vi "snapPoint.vi"(0 "reference":refnum<class "Grid.lvclass">, 1 "point2D":T1 {"y" format="%.2f"; "x" format="%.2f"}, 5 "error in (no error)":errorcluster) -> (14 "reference out":refnum<class "Grid.lvclass">, 15 "point2D 2":T1 {"y" format="%.2f"; "x" format="%.2f"}, 19 "error out":errorcluster)   [LabVIEW 2020, in "Grid.lvclass"]
doc: "public void snap(Point2D p)"
uses:
  <resource>/Framework/Providers/Open_GDS/UML/Grid_class/Grid.lvclass
  <resource>/Framework/Providers/Open_GDS/UML/General/Point/Point Point2D.ctl
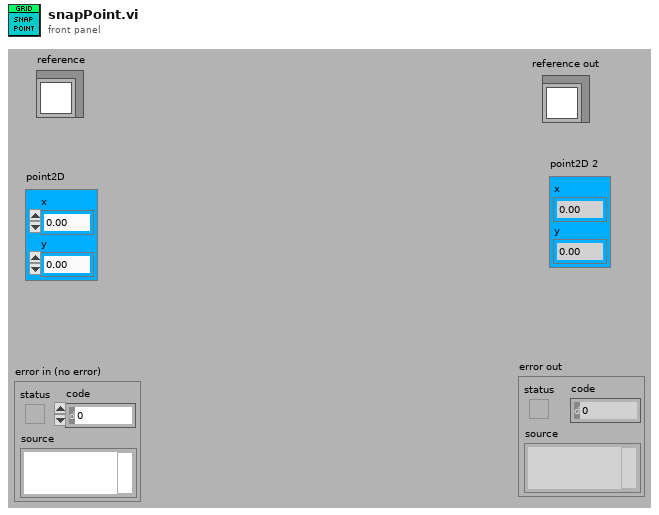
[diagram p1: front panel]
types:
  T1 = typedef "Point Point2D.ctl" = cluster{"x":dbl, "y":dbl}
  T2 = typedef "Grid.lvclass/ObjectAttributes.ctl" = cluster{"gridX":dbl, "gridY":dbl, "gridColor":u32}
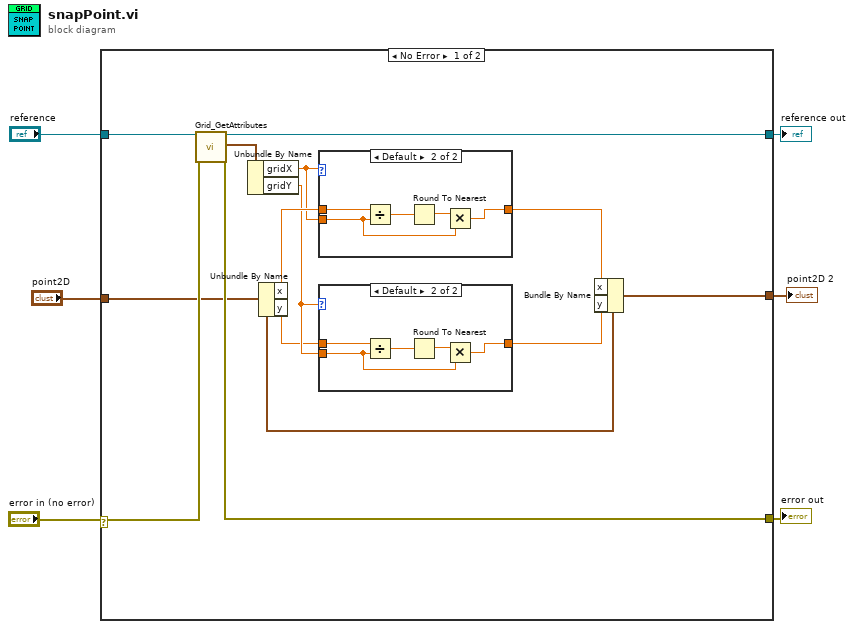
[diagram p0: block diagram]
diagram:
  n1 = case shown="No Error" "error in (no error)" {
    selector: "error in (no error)" -> [w16 w32]
    tunnel: "reference" -> [w19 w33]
    tunnel: [w18 w32] -> w5
    tunnel: [w17 w33] -> w4
    tunnel: "point2D" -> [w15 _]
    tunnel: [w14 _] -> w1
    frame No Error {
      n2 = call <resource>:"Grid_GetAttributes.vi"("reference in"=w19, "error in (no error)"=w16) -> ("reference out"=w17:refnum<class "Grid.lvclass">, "Data"=w7:T2, "error out"=w18:errorcluster)  [unwired: 1 in, 14 out]
      n3 = Unbundle By Name(w7) -> ("gridX"=w12:dbl, "gridY"=w10:dbl)
      n4 = Unbundle By Name(w15) -> ("x"=w13:dbl, "y"=w9:dbl)
      n5 = case shown="Default" w12 {
        tunnel: w13 -> [w26 w31]
        tunnel: w12 -> [_ w28]
        tunnel: [w26 w27] -> w11
        frame 0 {
        }
        frame Default {
          n6 = Divide(x=w31, y=w28) -> (x/y=w30:dbl)
          n7 = Round To Nearest(number=w30) -> (nearest integer value=w29:dbl)
          n8 = Multiply(x=w29, y=w28) -> (x*y=w27:dbl)
        }
      }
      n9 = case shown="Default" w10 {
        tunnel: w9 -> [w20 w25]
        tunnel: w10 -> [_ w22]
        tunnel: [w20 w21] -> w8
        frame 0 {
        }
        frame Default {
          n10 = Divide(x=w25, y=w22) -> (x/y=w24:dbl)
          n11 = Round To Nearest(number=w24) -> (nearest integer value=w23:dbl)
          n12 = Multiply(x=w23, y=w22) -> (x*y=w21:dbl)
        }
      }
      n13 = Bundle By Name(cluster=w15, "x"=w11, "y"=w8) -> (w14:T1)
    }
    frame Error {
    }
  }
  "reference out" <- w4
  "error out" <- w5
  "point2D 2" <- w1
